vi "Log.vi"   [LabVIEW 2018, in "GLog.lvlib" / "Logger.lvclass"]
uses:
  Logger.lvclass
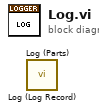
[diagram p0: block diagram]
diagram:
  n1 = call "Log (Log Record).vi"() -> ()  [unwired: 11 in, 1 out]
  n2 = call "Log (Parts).vi"() -> ()  [unwired: 11 in, 1 out]
